vi "Replace Line.vi"(8 "error in":errorcluster, 9 "New Line":T1, 10 "Line Name":string, 11 "Shared Memory configuration in":refnum<class "Shared Memory configuration.lvclass">) -> (0 "error out":errorcluster, 2 "Old Line":T1, 3 "Shared Memory configuration out":refnum<class "Shared Memory configuration.lvclass">)   [LabVIEW 2014, in "Shared Memory configuration.lvclass"]
doc: "Replaces a line identified by name with a new line."
uses:
  Shared Memory configuration.lvclass
  Line.ctl
  <vilib>/NI/Tag Bus Module Framework/channel/TBM channel.lvclass
  Shared Memory configuration.lvclass/Shared Memory configuration.ctl
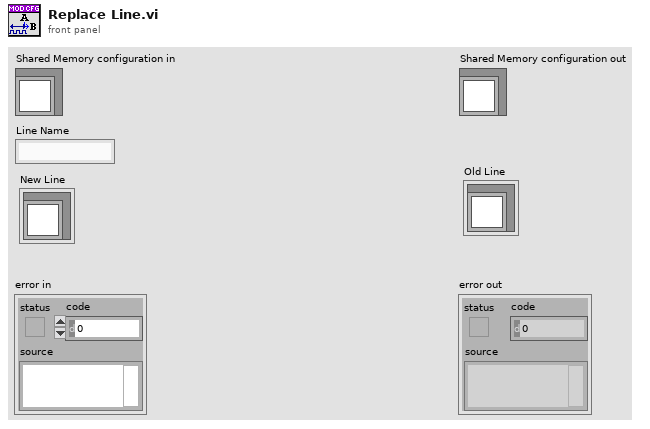
[diagram p1: front panel]
types:
  T1 = typedef "Shared Memory configuration.lvclass/Line.ctl" = cluster{"channel":refnum<class "TBM channel.lvclass">}
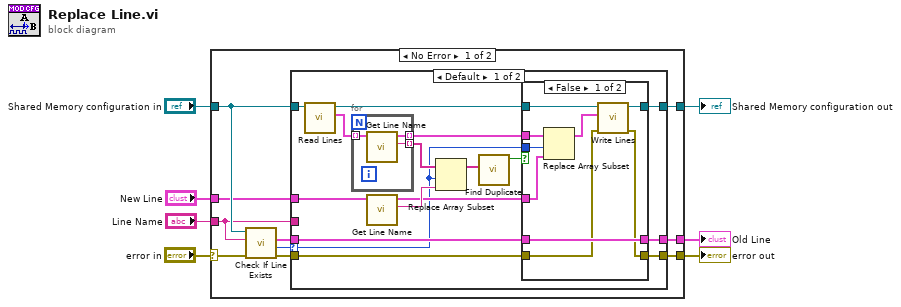
[diagram p0: block diagram]
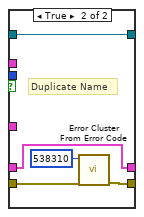
[diagram p2: hidden frame]
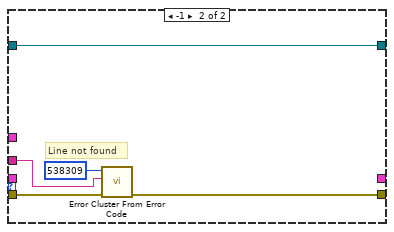
[diagram p3: hidden frame]
diagram:
  n1 = case shown="No Error" "error in" {
    selector: "error in" -> [w10 w57]
    tunnel: [w16 w57] -> w6
    tunnel: [w17 w56] -> w4
    tunnel: "Shared Memory configuration in" -> [w15 w56]
    tunnel: "Line Name" -> [w14 _]
    tunnel: "New Line" -> [w12 _]
    tunnel: [w11 _] -> w1
    frame No Error {
      n2 = call-dynamic "Check If Line Exists.vi"("error in"=w10, "Name to Locate"=w14, "Shared Memory configuration in"=w15) -> ("error out"=w9:errorcluster, "Index"=w13:i32, "Line out"=w8:T1)  [unwired: 4 in, 2 out]
      n3 = case shown="Default" w13 {
        selector: w13 -> [w19 _]
        tunnel: w15 -> [w33 w55]
        tunnel: [w25 w55] -> w17
        tunnel: w12 -> [w30 _]
        tunnel: w14 -> [_ w53]
        tunnel: w9 -> [w24 w52]
        tunnel: [w23 w51] -> w16
        tunnel: [w22 _] -> w11
        tunnel: w8 -> [w21 _]
        frame Default {
          n4 = call "Read Lines.vi"("Shared Memory configuration in"=w33) -> ("Lines"=w32:T1[], "Shared Memory configuration out"=w26:refnum<class "Shared Memory configuration.lvclass">)  [unwired: 8 in, 1 out]
          n5 = for {
            tunnel: w32 -> [w50] mode=indexing
            tunnel: [w49] -> w28 mode=indexing
            tunnel: [w48] -> w31 mode=indexing
            n6 = call "Get Line Name.vi"("Line in"=w50) -> ("Name"=w48:string, "Line out"=w49:T1)  [unwired: 8 in, 1 out]
          }
          n7 = call "Get Line Name.vi"("Line in"=w30) -> ("Name"=w29:string, "Line out"=w20:T1)  [unwired: 8 in, 1 out]
          n8 = Replace Array Subset(array=w31, new element=w29, index=w19) -> (w27:string[])
          n9 = call "Find Duplicate.vi"("Array"=w27) -> ("Duplicate"=w18:bool)  [unwired: 8 in, 2 out]
          n10 = case shown="False" w18 {
            tunnel: w28 -> [w42 _]
            tunnel: w26 -> [w38 w47]
            tunnel: [w37 w47] -> w25
            tunnel: w24 -> [w35 w46]
            tunnel: [w34 w45] -> w23
            tunnel: [w41 w44] -> w22
            tunnel: w21 -> [w41 w44]
            tunnel: w20 -> [w40 _]
            tunnel: w19 -> [w36 _]
            frame False {
              n11 = Replace Array Subset(array=w42, new element=w40, index=w36) -> (w39:T1[])
              n12 = call "Write Lines.vi"("error in (no error)"=w35, "Lines"=w39, "Shared Memory configuration in"=w38) -> ("error out"=w34:errorcluster, "Shared Memory configuration out"=w37:refnum<class "Shared Memory configuration.lvclass">)  [unwired: 7 in]
            }
            frame True {
              # "Duplicate Name"
              n13 = call <vilib>:"Error Cluster From Error Code.vi"("error in (no error)"=w46, "error code (0)"=538310) -> ("error out"=w45:errorcluster)  [unwired: 7 in]
            }
          }
        }
        frame -1 {
          # "Line not found"
          n14 = call <vilib>:"Error Cluster From Error Code.vi"("error in (no error)"=w52, "error message (\"\")"=w53, "error code (0)"=538309) -> ("error out"=w51:errorcluster)  [unwired: 6 in]
        }
      }
    }
    frame Error {
    }
  }
  "error out" <- w6
  "Shared Memory configuration out" <- w4
  "Old Line" <- w1
